vi "Replace Line.vi"(8 "error in":errorcluster, 9 "New Line":T1 {"OPC UA Data Type" items=["Boolean"=1, "SByte"=2, "Byte"=3, "Int16"=4, "UInt16"=5, "Int32"=6, "UInt32"=7, "Int64"=8, "UInt64"=9, "Float"=10, "Double"=11, "String"=12, "DateTime"=13, "ByteString"=15, "Array of Boolean"=101, "Array of SByte"=102, "Array of Byte"=103, "Array of Int16"=104, "Array of UInt16"=105, "Array of Int32"=106, "Array of UInt32"=107, "Array of Int64"=108, "Array of UInt64"=109, "Array of Float"=110, "Array of Double"=111, "Array of String"=112, "Array of DateTime"=113, "Array of ByteString"=115]}, 10 "Line Name":string, 11 "OPC UA configuration in":refnum<class "OPC UA Client configuration.lvclass">) -> (0 "error out":errorcluster, 2 "Old Line":T1 {"OPC UA Data Type" items=["Boolean"=1, "SByte"=2, "Byte"=3, "Int16"=4, "UInt16"=5, "Int32"=6, "UInt32"=7, "Int64"=8, "UInt64"=9, "Float"=10, "Double"=11, "String"=12, "DateTime"=13, "ByteString"=15, "Array of Boolean"=101, "Array of SByte"=102, "Array of Byte"=103, "Array of Int16"=104, "Array of UInt16"=105, "Array of Int32"=106, "Array of UInt32"=107, "Array of Int64"=108, "Array of UInt64"=109, "Array of Float"=110, "Array of Double"=111, "Array of String"=112, "Array of DateTime"=113, "Array of ByteString"=115]}, 3 "OPC UA configuration out":refnum<class "OPC UA Client configuration.lvclass">)   [LabVIEW 2014, in "OPC UA Client configuration.lvclass"]
uses:
  OPC UA Client configuration.lvclass
  Line.ctl
  <vilib>/NI/Tag Bus Module Framework/channel/TBM channel.lvclass
  OPC UA Data Type.ctl
  OPC UA Client configuration.lvclass/OPC UA Client configuration.ctl
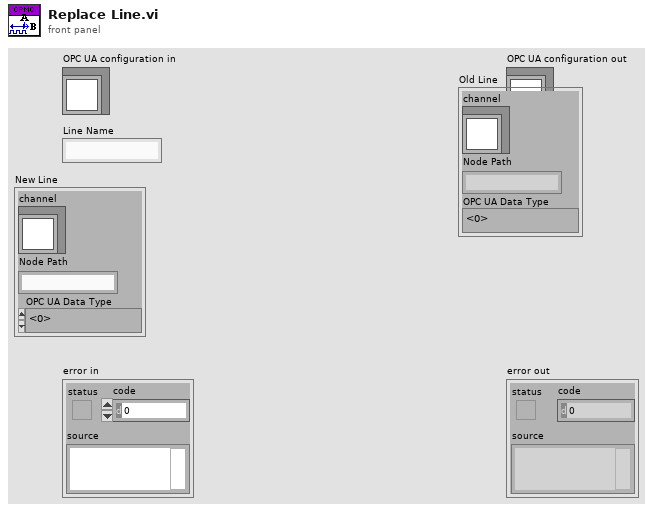
[diagram p1: front panel]
types:
  T1 = typedef "OPC UA Client configuration.lvclass/Line.ctl" = cluster{"channel":refnum<class "TBM channel.lvclass">, "Node Path":string, "OPC UA Data Type":T2}
  T2 = typedef "OPC UA Client configuration.lvclass/OPC UA Data Type.ctl" = u16
  T3 = cluster{"channel":refnum<class "TBM channel.lvclass">, "Node Path":string, "OPC UA Data Type":T2}[]
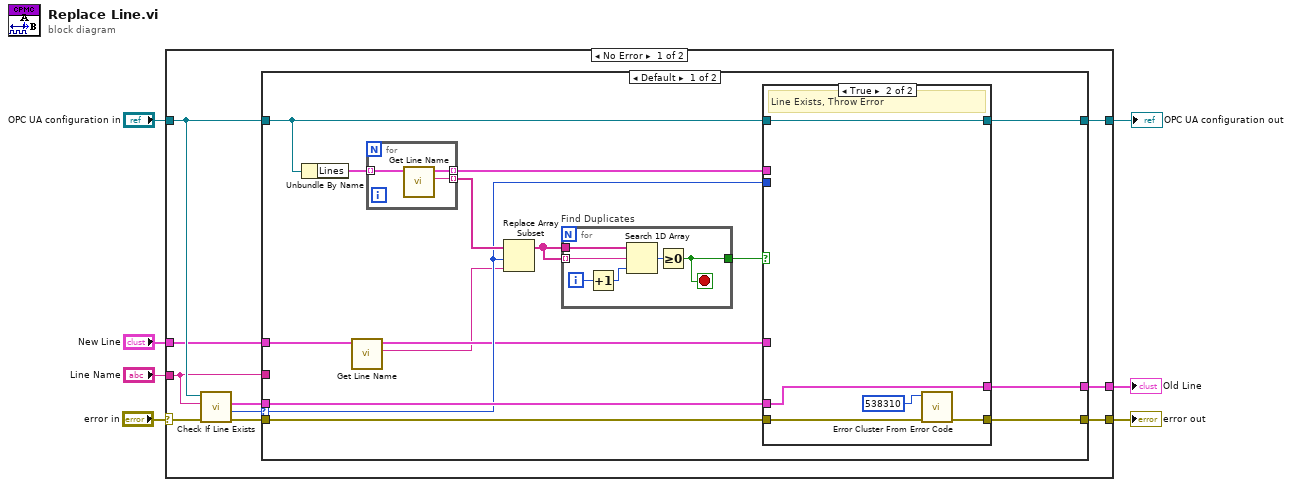
[diagram p0: block diagram]
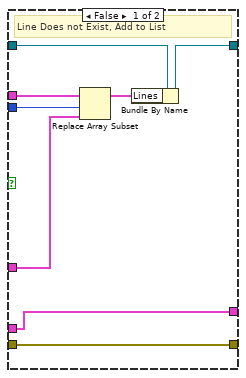
[diagram p2: hidden frame]
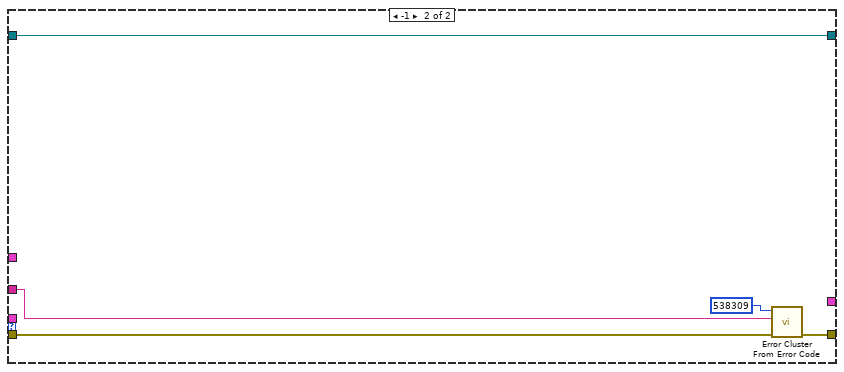
[diagram p3: hidden frame]
diagram:
  n1 = case shown="No Error" "error in" {
    selector: "error in" -> [w10 w61]
    tunnel: [w16 w61] -> w6
    tunnel: [w17 w60] -> w4
    tunnel: "OPC UA configuration in" -> [w15 w60]
    tunnel: "Line Name" -> [w14 _]
    tunnel: "New Line" -> [w12 _]
    tunnel: [w11 _] -> w1
    frame No Error {
      n2 = call-dynamic "Check If Line Exists.vi"("error in"=w10, "name to locate"=w14, "OPC UA configuration in"=w15) -> ("error out"=w9:errorcluster, "index"=w13:i32, "Line out"=w8:T1)  [unwired: 4 in, 2 out]
      n3 = case shown="Default" w13 {
        selector: w13 -> [w22 _]
        tunnel: w15 -> [w30 w59]
        tunnel: [w32 w59] -> w17
        tunnel: w12 -> [w31 _]
        tunnel: w14 -> [_ w57]
        tunnel: w9 -> [w28 w56]
        tunnel: [w27 w55] -> w16
        tunnel: [w25 _] -> w11
        tunnel: w8 -> [w26 _]
        frame Default {
          n4 = Unbundle By Name(w30) -> ("Lines"=w29:T3)
          n5 = call "Get Line Name.vi"("Line in"=w31) -> ("Name"=w20:string, "Line out"=w21:T1)  [unwired: 8 in, 1 out]
          n6 = for {
            tunnel: w29 -> [w54] mode=indexing
            tunnel: [w53] -> w24 mode=indexing
            tunnel: [w52] -> w23 mode=indexing
            n7 = call "Get Line Name.vi"("Line in"=w54) -> ("Name"=w52:string, "Line out"=w53:T1)  [unwired: 8 in, 1 out]
          }
          n8 = Replace Array Subset(array=w23, new element=w20, index=w22) -> (w19:string[])
          n9 = for "Find Duplicates" {
            tunnel: w19 -> [w36]
            tunnel: w19 -> [w35] mode=indexing
            tunnel: [w33] -> w18
            i -> [w38]
            stop <- w33 stop-if-true
            n10 = Increment(x=w38) -> (x+1=w37:i32)
            n11 = Search 1D Array(1D array=w36, element=w35, start index (0)=w37) -> (index of element=w34:i32)
            n12 = Greater Or Equal To 0?(x=w34) -> (x >= 0?=w33:bool)
          }
          n13 = case shown="True" w18 {
            tunnel: [w39 w51] -> w32
            tunnel: w21 -> [w45 _]
            tunnel: w30 -> [w44 w51]
            tunnel: w28 -> [w43 w49]
            tunnel: [w43 w48] -> w27
            tunnel: w26 -> [w42 w50]
            tunnel: [w42 w50] -> w25
            tunnel: w24 -> [w40 _]
            tunnel: w22 -> [w41 _]
            frame False {
              # "Line Does not Exist, Add to List"
              n14 = Replace Array Subset(array=w40, new element=w45, index=w41) -> (w46:T1[])
              n15 = Bundle By Name(cluster=w44, "Lines"=w46) -> (w39:refnum<class "OPC UA Client configuration.lvclass">)
            }
            frame True {
              # "Line Exists, Throw Error"
              n16 = call <vilib>:"Error Cluster From Error Code.vi"("error in (no error)"=w49, "error code (0)"=538310) -> ("error out"=w48:errorcluster)  [unwired: 7 in]
            }
          }
        }
        frame -1 {
          n17 = call <vilib>:"Error Cluster From Error Code.vi"("error in (no error)"=w56, "error message (\"\")"=w57, "error code (0)"=538309) -> ("error out"=w55:errorcluster)  [unwired: 6 in]
        }
      }
    }
    frame Error {
    }
  }
  "error out" <- w6
  "OPC UA configuration out" <- w4
  "Old Line" <- w1
